vi "App_Close.vi"(0 "Channels":T1, 11 "error in":errorcluster) -> (15 "error out":errorcluster)   [LabVIEW 2020, in "GH_App.lvlib"]
doc: "End of Main (after the engine and picture loops): releases the queues and the notifier; the audio loop ends because its queue is gone. Errors of the loops come in through error in and are kept."
uses:
  GH_App.lvlib
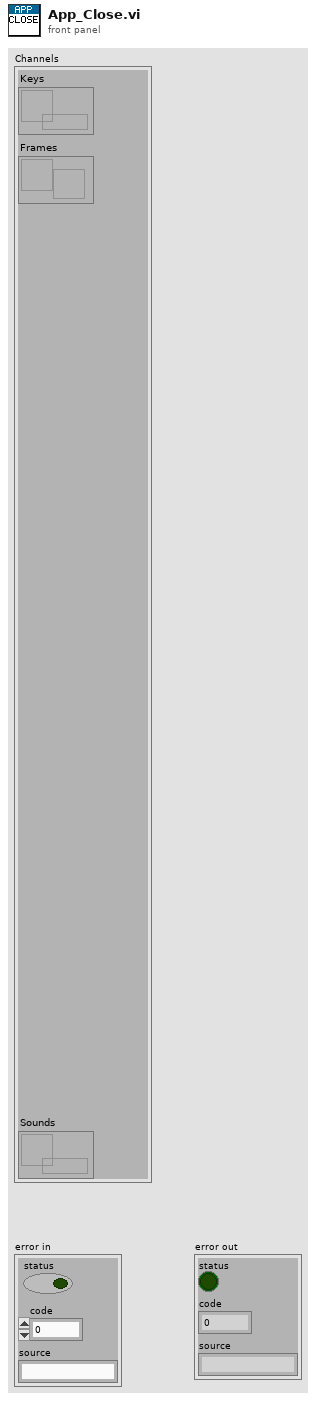
[diagram p1: front panel]
types:
  T1 = cluster{"Keys":refnum<queue>, "Frames":refnum<notifier>, "Sounds":refnum<queue>}
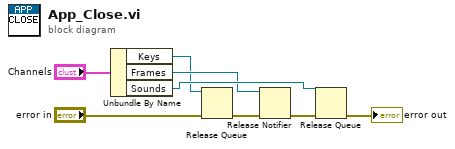
[diagram p0: block diagram]
diagram:
  n1 = Unbundle By Name("Channels") -> ("Keys"=w3:refnum<queue>, "Frames"=w4:refnum<notifier>, "Sounds"=w5:refnum<queue>)
  n2 = Release Queue(queue=w3, error in (no error)="error in") -> (error out=w6:errorcluster)  [unwired: 1 in, 2 out]
  n3 = Release Notifier(notifier=w4, error in (no error)=w6) -> (error out=w7:errorcluster)  [unwired: 1 in, 2 out]
  n4 = Release Queue(queue=w5, error in (no error)=w7) -> (error out=→"error out":errorcluster)  [unwired: 1 in, 2 out]
